vi "RTM SLSC Autodetect.vi"(8 "error in (no error)":errorcluster, 11 "Node Ptr":T1=18446744073709551615 format="%.0x") -> (0 "error out":errorcluster)   [LabVIEW 2020, in "SLSC EDS System Explorer.lvlib"]
uses:
  SLSC EDS System Explorer.lvlib
  <vilib>/NI VeriStand/Custom Device API/Custom Device Item Ref.ctl
  <vilib>/NI VeriStand/Custom Device Tools/Custom Device Utility Library/Custom Device Utility Library.lvlib
  <vilib>/NI VeriStand/Custom Device API/Custom Device API.lvlib
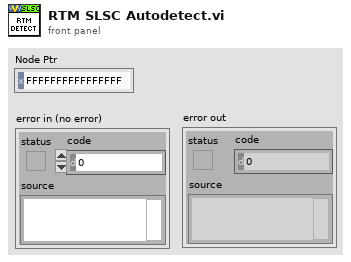
[diagram p1: front panel]
types:
  T1 = typedef "Custom Device API.lvlib/Custom Device Item Ref.ctl" = u64
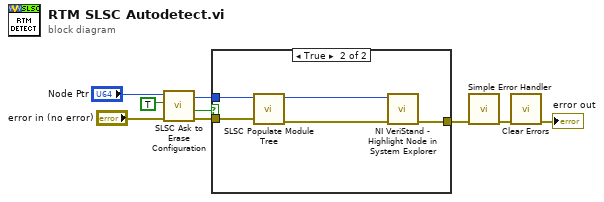
[diagram p0: block diagram]
diagram:
  n1 = call "SLSC Ask to Erase Configuration.vi"("error in (no error)"="error in (no error)", "Ask to erase?"=TRUE, "Device Item Ref in"="Node Ptr") -> ("error out"=w3:errorcluster, "Erase Data?"=w2:bool, "Item Ref out"=w1:T1)  [unwired: 5 in, 1 out]
  n2 = case shown="True" w2 {
    tunnel: [w10 w14] -> w7
    tunnel: w3 -> [w10 w13]
    tunnel: w1 -> [_ w12]
    frame False {
    }
    frame True {
      n3 = call "SLSC Populate Module Tree.vi"("error in (no error)"=w13, "Device Item Ref in"=w12) -> ("error out"=w11:errorcluster, "Device Item Ref out"=w15:T1)  [unwired: 5 in, 3 out]
      n4 = call <vilib>:"NI VeriStand - Highlight Node in System Explorer.vi"("error in (no error)"=w11, "Item Ref in"=w15) -> ("error out"=w14:errorcluster)  [unwired: 8 in, 1 out]
    }
  }
  n5 = call <vilib>:"Simple Error Handler.vi"("error in (no error)"=w7) -> ("error out"=w9:errorcluster)  [unwired: 4 in, 4 out]
  n6 = call <vilib>:"Clear Errors.vi"("error in (no error)"=w9) -> ("error out"=→"error out":errorcluster)  [unwired: 5 in, 1 out]
